vi "Dequeue Byte.vi"(8 "error in":errorcluster, 9 "error if not found?":bool=TRUE caption="error if not found? (T)", 11 "Buffer":refnum<data-value>) -> (0 "error out":errorcluster, 1 "found":bool, 2 "byte":u8 format="%02x", 3 "Buffer":refnum<data-value>, 4 "buffer empty?":bool)   [LabVIEW 2013, in "CircularBuffer.lvlib" / "ByteFIFO.lvclass"]
doc: "This VI allows to input an array into the buffer. The location in the buffer is updated automatically.\n\nIf the input array is larger than the buffer then just take last elements of the input array and save them in the buffer. Also give a warning that this happened."
uses:
  ByteFIFO.lvclass
  VariantBuffer/VariantBuffer.lvclass
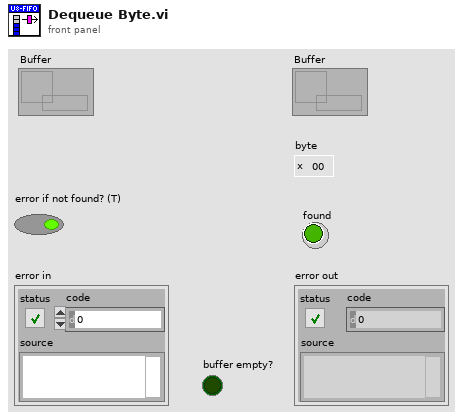
[diagram p1: front panel]
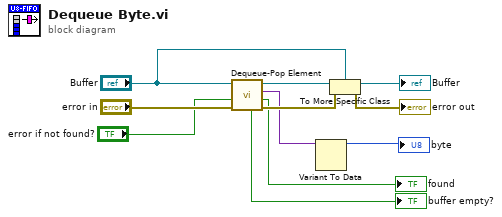
[diagram p0: block diagram]
diagram:
  n1 = call "Dequeue-Pop Element.vi"("error in"="error in", "error if not found?"="error if not found?", "Buffer in"="Buffer") -> ("error out"=w5:errorcluster, "found"=→"found":bool, "element"=w4:variant, "Buffer"=w7:refnum<data-value>, "buffer empty?"=→"buffer empty?":bool)  [unwired: 4 in]
  n2 = Variant To Data(Variant=w4) -> (data=→"byte":u8)  [unwired: 2 in, 1 out]
  n3 = To More Specific Class(target class="Buffer", reference=w7, error in=w5) -> (specific class reference=→"Buffer":refnum<data-value>, error out=→"error out":errorcluster)
